vi "SQL_Connection-Name.vi"(4 "Passwort":string, 6 "User Name":string, 8 "error in (no error)":errorcluster caption="Fehler (Eingang, kein Fehler)", 9 "Database Name":string, 10 "Server Name":string, 11 "SQL Driver  Clientname":string) -> (0 "error out":errorcluster caption="Fehler (Ausgang)", 3 "Connection String":string)   [LabVIEW 2024, in "DB-Tool.lvlib"]
doc: "<b>Connectionstring - Windows User</b>\nProvider=<b>SQLclient</b>;\nIntegrated Security=SSPI;\nPersist Security Info=false;\nData Source=<b>TestServer</b>;\nInitial Catalog=<b>TestDB</b>\n\n<b>Connectionstring - Definied User (e.g. Global DB in Azure)</b>\nProvider=<b>SQLclient</b>;\nPersist Security Info=false;\nData Source=<b>TestServer</b>;\nInitial Catalog=<b>TestDB</b>;\nUser Id=\"<b>Usertest</b>\";\nPassword=\"<b>Userpassword</b>\""
uses:
  DB-Tool.lvlib
  <vilib>/Utility/error.llb/Trim Whitespace One-Sided.vi
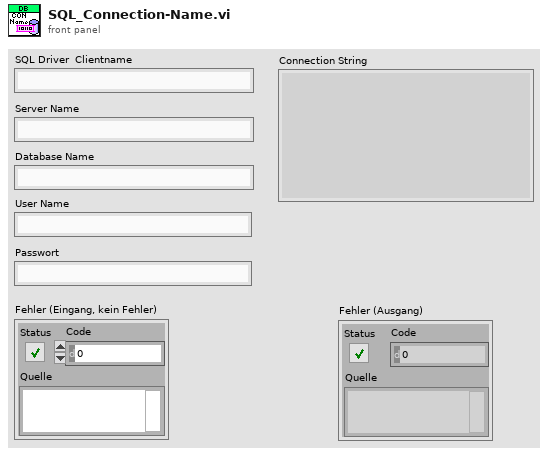
[diagram p1: front panel]
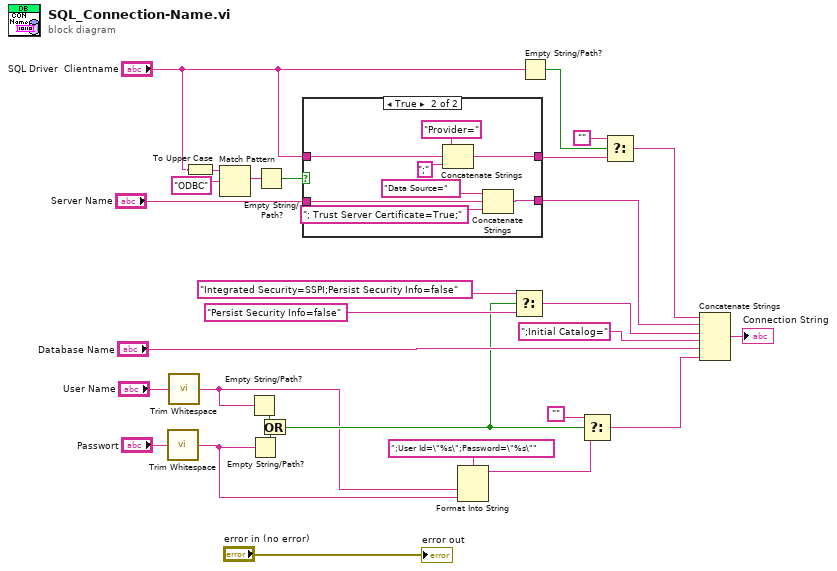
[diagram p0: block diagram]
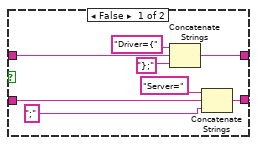
[diagram p2: hidden frame]
diagram:
  n1 = call <vilib>:"Trim Whitespace.vi"("string"="Passwort") -> ("trimmed string"=w14:string)  [unwired: 1 in]
  n2 = call <vilib>:"Trim Whitespace.vi"("string"="User Name") -> ("trimmed string"=w15:string)  [unwired: 1 in]
  n3 = To Upper Case(1:"SQL Driver  Clientname") -> (0:w9:string)
  n4 = Match Pattern(string=w9, regular expression="ODBC") -> (match substring=w12:string)  [unwired: 1 in, 3 out]
  n5 = Empty String/Path?(string/path=w15) -> (empty?=w28:bool)
  n6 = Empty String/Path?(string/path=w14) -> (empty?=w27:bool)
  n7 = Empty String/Path?(string/path=w12) -> (empty?=w10:bool)
  n8 = Or(x=w28, y=w27) -> (x .or. y?=w16:bool)
  n9 = case shown="True" w10 {
    tunnel: "SQL Driver  Clientname" -> [w36 w44]
    tunnel: [w34 w42] -> w7
    tunnel: [w31 w39] -> w2
    tunnel: "Server Name" -> [w32 w40]
    frame False {
      n10 = Concatenate Strings("Driver={", w36, "};") -> (w34:string)
      n11 = Concatenate Strings("Server=", w32, ";") -> (w31:string)
    }
    frame True {
      n12 = Concatenate Strings("Provider=", w44, ";") -> (w42:string)
      n13 = Concatenate Strings("Data Source=", w40, "; Trust Server Certificate=True;") -> (w39:string)
    }
  }
  n14 = Format Into String(format string=";User Id=\"%s\";Password=\"%s\"", w15, w14) -> (resulting string=w19:string)  [unwired: 2 in, 1 out]
  n15 = Select(t="Integrated Security=SSPI;Persist Security Info=false", s=w16, f="Persist Security Info=false") -> (s? t:f=w1:string)
  n16 = Empty String/Path?(string/path="SQL Driver  Clientname") -> (empty?=w3:bool)
  n17 = Select(t="", s=w16, f=w19) -> (s? t:f=w13:string)
  n18 = Select(t="", s=w3, f=w7) -> (s? t:f=w5:string)
  n19 = Concatenate Strings(w5, w2, w1, ";Initial Catalog=", "Database Name", w13) -> (→"Connection String":string)
  "error out" <- "error in (no error)"
